vi "Valued.vi"(10 "单元格位置":cluster{"Row":i32, "Column":i32}, 11 "数组":string[][](array[string])) -> (3 "元素":string)   [LabVIEW 2025]
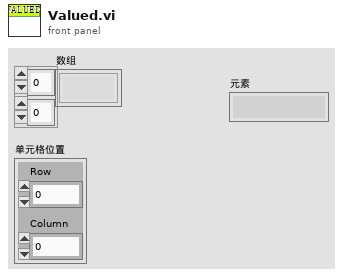
[diagram p1: front panel]
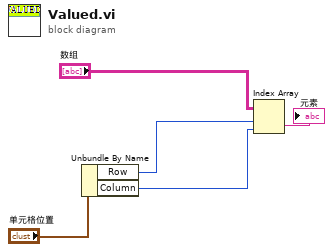
[diagram p0: block diagram]
diagram:
  n1 = Unbundle By Name("单元格位置") -> ("Row"=w3:i32, "Column"=w2:i32)
  n2 = Index Array(array="数组", index (row)=w3, index (col)=w2) -> (element=→"元素":string)
